vi "WriteSuccessFile.vi"(8 "error in (no error)":errorcluster, 9 "Generated file":T1, 11 "SolutionBuilder in":refnum<class "SolutionBuilder.lvclass">) -> (0 "error out":errorcluster, 3 "SolutionBuilder out":refnum<class "SolutionBuilder.lvclass">)   [LabVIEW 2019, in "SolutionBuilder.lvlib" / "SolutionBuilder.lvclass"]
uses:
  SolutionBuilder.lvclass
  BuildManager/GeneratedFile.ctl
  BuildManager/BuildManager.lvclass
  BuildManager/BuildProjectInfo.ctl
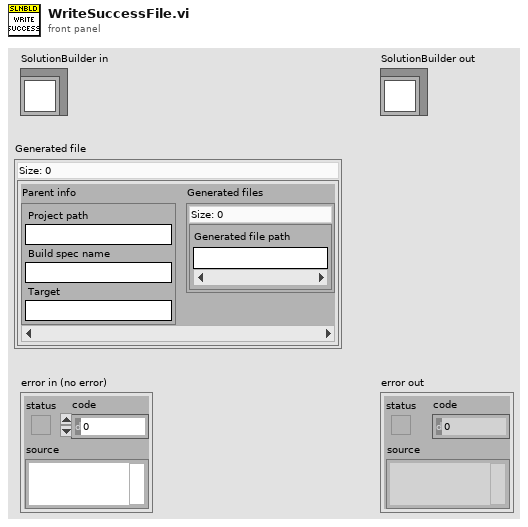
[diagram p1: front panel]
types:
  T1 = typedef "SolutionBuilder.lvlib/BuildManager.lvclass/GeneratedFile.ctl" = map{T2, set{string}}
  T2 = typedef "SolutionBuilder.lvlib/BuildManager.lvclass/BuildProjectInfo.ctl" = cluster{"Project path":string, "Build spec name":string, "Target":string}
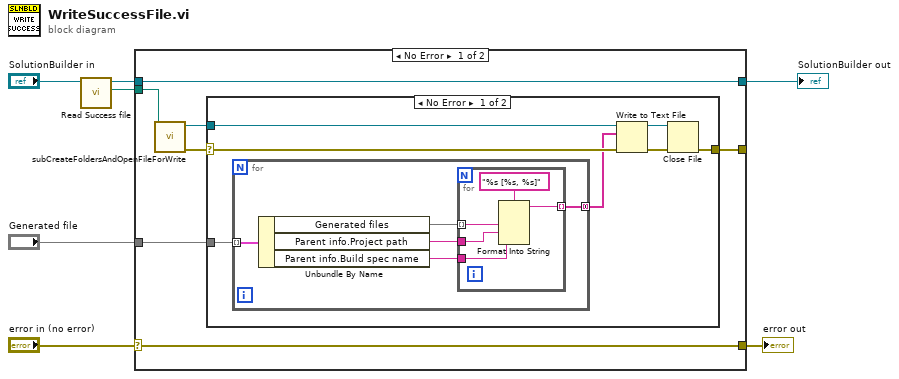
[diagram p0: block diagram]
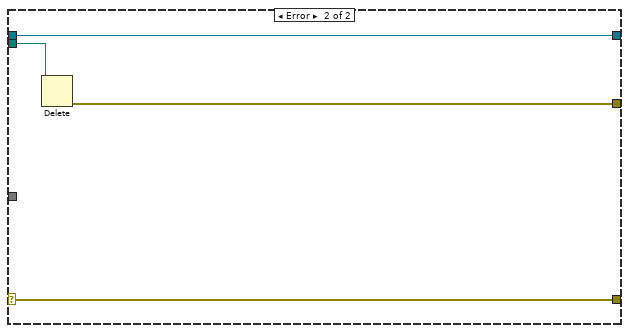
[diagram p3: hidden frame]
diagram:
  n1 = call "Read Success file.vi"("SolutionBuilder in"="SolutionBuilder in") -> ("Success file"=w2:path, "SolutionBuilder out"=w3:refnum<class "SolutionBuilder.lvclass">)  [unwired: 9 in]
  n2 = case shown="No Error" "error in (no error)" {
    selector: "error in (no error)" -> [w14 w35]
    tunnel: [w14 w35] -> w6
    tunnel: [w9 w34] -> w5
    tunnel: w3 -> [w9 w34]
    tunnel: "Generated file" -> [w11 _]
    tunnel: w2 -> [w10 w33]
    tunnel: [w8 w32] -> _
    frame No Error {
      n3 = call "subCreateFoldersAndOpenFileForWrite.vi"("File path"=w10) -> ("error out"=w13:errorcluster, "File ref"=w12:refnum<file>)  [unwired: 9 in]
      n4 = case shown="No Error" w13 {
        selector: w13 -> [w20 _]
        tunnel: w12 -> [w21 _]
        tunnel: w11 -> [w19 _]
        tunnel: [w15 _] -> w8
        frame No Error {
          n5 = for {
            tunnel: w19 -> [w25] mode=indexing
            tunnel: [w26] -> w18 mode=concatenating
            n6 = Unbundle By Name(w25) -> ("Generated files"=w23:set{string}, "Parent info.Project path"=w22:string, "Parent info.Build spec name"=w24:string)
            n7 = for {
              tunnel: [w30] -> w26 mode=indexing
              tunnel: w24 -> [w29]
              tunnel: w23 -> [w28] mode=indexing
              tunnel: w22 -> [w27]
              n8 = Format Into String(format string="%s [%s, %s]", w28, w27, w29) -> (resulting string=w30:string)  [unwired: 2 in, 1 out]
            }
          }
          n9 = Write to Text File(file (use dialog)=w21, text=w18, error in=w20) -> (refnum out=w17:refnum<file>, error out=w16:errorcluster)  [unwired: 1 in, 1 out]
          n10 = Close File(refnum=w17, error in=w16) -> (error out=w15:errorcluster)  [unwired: 1 out]
        }
        frame Error {
        }
      }
    }
    frame Error {
      n11 = Delete(path (use dialog)=w33) -> (error out=w32:errorcluster)  [unwired: 4 in, 2 out]
    }
  }
  "error out" <- w6
  "SolutionBuilder out" <- w5
